vi "set Swept SA - Marker Auto Search Type.vi"(6 "Auto Search On?":bool, 8 "error in (no error)":errorcluster, 9 "Index":i32, 10 "Marker Auto Type":T1, 11 "FSV-40N in":refnum<class "FSV-40N.lvclass">) -> (0 "error out":errorcluster, 3 "FSV-40N out":refnum<class "FSV-40N.lvclass">)   [LabVIEW 2023, in "Spectrum Analyzer.lvlib" / "FSV-40N.lvclass"]
uses:
  FSV-40N.lvclass
  FSV-40N.lvclass/FSV-40N.ctl
  <vilib>/ErrorRing/Error Ring.xnode
  TYPE DEFINITION/TYPE Marker Auto Select.ctl
  Spectrum Analyzer.lvlib
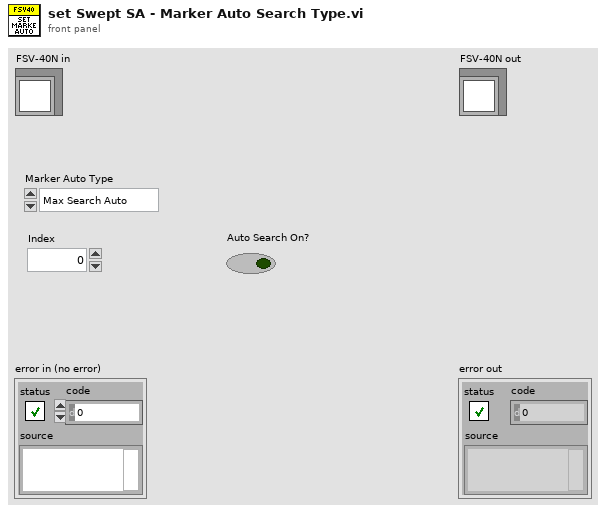
[diagram p1: front panel]
types:
  T1 = typedef "Spectrum Analyzer.lvlib/TYPE Marker Auto Select.ctl" = enum16{"Max Search Auto", "Min Search Auto"}
  T2 = typedef "Spectrum Analyzer.lvlib/TYPE Marker Type Map.ctl" = map{i32, T3}
  T3 = typedef "Spectrum Analyzer.lvlib/TYPE Marker Control Mode.ctl" = enum16{"Normal", "Delta", "Off"}
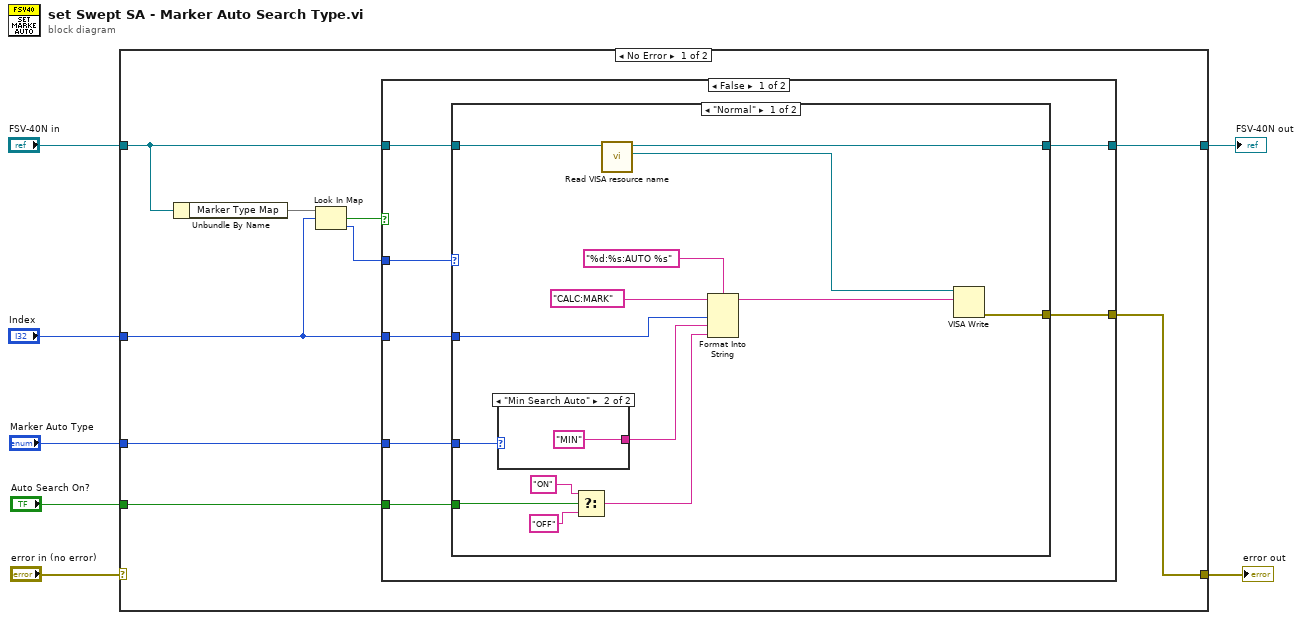
[diagram p0: block diagram]
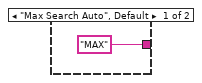
[diagram p2: hidden frame]
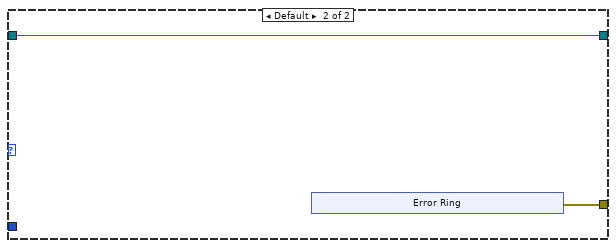
[diagram p3: hidden frame]
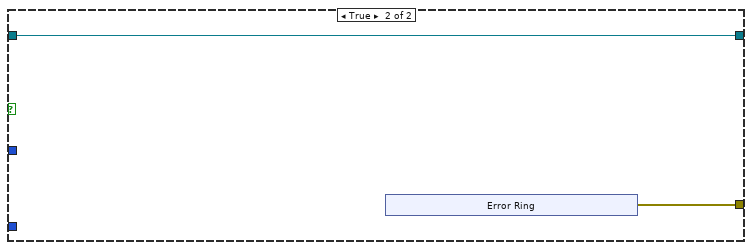
[diagram p4: hidden frame]
diagram:
  n1 = case shown="No Error" "error in (no error)" {
    selector: "error in (no error)" -> [_ w46]
    tunnel: "FSV-40N in" -> [w13 w47]
    tunnel: [w14 w47] -> w5
    tunnel: [w15 w46] -> w4
    tunnel: "Marker Auto Type" -> [w16 _]
    tunnel: "Index" -> [w11 _]
    tunnel: "Auto Search On?" -> [w8 _]
    frame No Error {
      n2 = Unbundle By Name(w13) -> ("Marker Type Map"=w12:T2)
      n3 = Look In Map(map=w12, key=w11) -> (key not found?=w10:bool, value=w9:T3)  [unwired: 1 in]
      n4 = case shown="False" w10 {
        tunnel: w16 -> [w23 _]
        tunnel: [w22 w43] -> w15
        tunnel: [w21 w44] -> w14
        tunnel: w13 -> [w20 w44]
        tunnel: w11 -> [w19 _]
        tunnel: w9 -> [w18 _]
        tunnel: w8 -> [w17 _]
        frame False {
          n5 = case shown="\"Normal\"" w18 {
            tunnel: w23 -> [w29 _]
            tunnel: [w36 w40] -> w22
            tunnel: [w35 w41] -> w21
            tunnel: w20 -> [w34 w41]
            tunnel: w19 -> [w31 _]
            tunnel: w17 -> [w27 _]
            frame "Normal" {
              n6 = case shown="\"Min Search Auto\"" w29 {
                tunnel: ["MAX" "MIN"] -> w30
                frame "Max Search Auto", Default {
                }
                frame "Min Search Auto" {
                }
              }
              n7 = Select(t="ON", s=w27, f="OFF") -> (s? t:f=w24:string)
              n8 = call "Read VISA resource name.vi"("FSV-40N in"=w34) -> ("VISA resource name"=w37:refnum<visa-resource-name>, "FSV-40N out"=w35:refnum<class "FSV-40N.lvclass">)  [unwired: 8 in, 1 out]
              n9 = Format Into String(format string="%d:%s:AUTO %s", initial string="CALC:MARK" ("string"), w31, w30, w24) -> (resulting string=w28:string)  [unwired: 1 in, 1 out]
              n10 = VISA Write(VISA resource name=w37, write buffer=w28) -> (error out=w36:errorcluster)  [unwired: 1 in, 2 out]
            }
            frame Default {
              n11 = xnode "Error Ring"() -> ("error out"=w40:errorcluster)
            }
          }
        }
        frame True {
          n12 = xnode "Error Ring"() -> ("error out"=w43:errorcluster)
        }
      }
    }
    frame Error {
    }
  }
  "error out" <- w4
  "FSV-40N out" <- w5
